vi "Format to Prometheus.vi"(8 "error in (no error)":errorcluster, 11 "Metric":refnum<data-value>) -> (0 "error out":errorcluster, 3 "Prometheus-formatted Metric":string[](array[string]))   [LabVIEW 2020, in "Metrics.lvlib" / "Metric.lvclass"]
uses:
  Metric.lvclass
  Metric.lvclass/Metric.ctl
  sample/Sample.lvclass
panel:
  out "Metric Out":refnum<data-value>
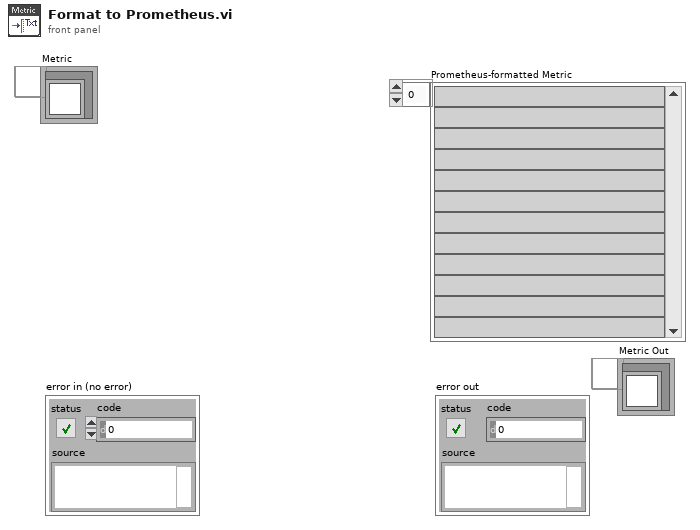
[diagram p1: front panel]
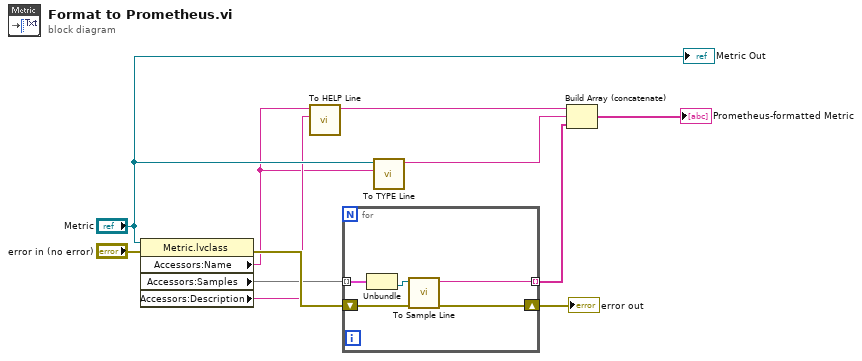
[diagram p0: block diagram]
diagram:
  n1 = property class="Metric.lvclass"(reference="Metric", error in="error in (no error)") -> (error out=w10:errorcluster, "Accessors:Name"=w5:string, "Accessors:Samples"=w8:map{string, refnum<class "Sample.lvclass">}, "Accessors:Description"=w6:string)  [unwired: 1 out]
  n2 = call "To HELP Line.vi"("Description"=w6, "Name"=w5) -> ("HELP line"=w4:string)  [unwired: 8 in, 1 out]
  n3 = for {
    tunnel: w8 -> [w13] mode=indexing
    tunnel: [w16] -> w2 mode=indexing
    shift-right: [w14] -> w11
    shift-left: w10 -> [w15]
    n4 = Unbundle(w13) -> (w12:refnum<class "Sample.lvclass">)  [unwired: 1 out]
    n5 = call "To Sample Line.vi"("error in (no error)"=w15, "Sample in"=w12) -> ("error out"=w14:errorcluster, "Sample line"=w16:string)  [unwired: 8 in]
  }
  "error out" <- w11
  n6 = call "To TYPE Line.vi"("Name"=w5, "Metric"="Metric") -> ("TYPE line"=w3:string)  [unwired: 8 in, 1 out]
  n7 = Build Array (concatenate)(w4, w3, w2) -> (→"Prometheus-formatted Metric":string[])
  "Metric Out" <- "Metric"
